vi "onTestDiscovery.vi"(8 "error in (no error)":errorcluster, 11 "Test Runner.Folder in":refnum<class "Test Runner.Folder.lvclass">) -> (0 "error out":errorcluster, 2 "Tests VIs":path[](array[path]), 3 "Test Runner.Folder out":refnum<class "Test Runner.Folder.lvclass">)   [LabVIEW 2020, in "Caraya.lvlib" / "Test Runner.Folder.lvclass"]
uses:
  Test Runner.Folder.lvclass
  Test Runner.Folder.lvclass/Test Runner.Folder.ctl
  <userlib>/_OpenG.lib/file/file.llb/openg_file.lvlib
  <userlib>/_OpenG.lib/file/file.llb/File Exists - Scalar__ogtk.vi
  Test Runner/Test Runner.lvclass
  <userlib>/_OpenG.lib/file/file.llb/Build Path - File Names Array__ogtk.vi
  <userlib>/_OpenG.lib/file/file.llb/File Exists - Array__ogtk.vi
  <userlib>/_OpenG.lib/file/file.llb/Valid Path - Traditional__ogtk.vi
  C:/projects/caraya/src/classes/Test Runner/Test Runner.lvclass
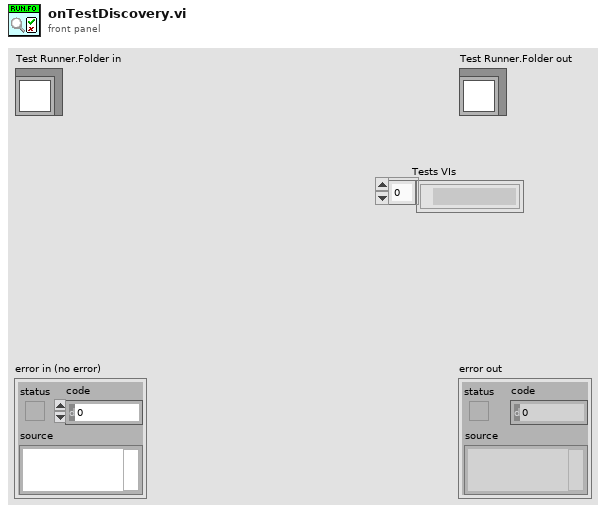
[diagram p1: front panel]
types:
  T1 = typedef "NI_FileType.lvlib/LVFileType.ctl" = enum32{"Invalid file", "Unknown type", "Instrument", "Control", "Polymorphic VI", "Project", "Library", "LVClass", "XControl", "XNode", "Shared library", ".NET assembly", "ActiveX interface", "CIN", "Run-time menu", "Palette menu", "Help file", "LLB", "XNode Edit Dependency", "Class Private Data Control", "Statechart", "MathScript .m file", "Ladder Diagram", "LVLibp", "XNode Build Dependency"}
  T2 = cluster{"path":path, "delimited name":string, "type":T1, "iState":u32, "iStyle":u16, "wStyle":u16, "buttons":u16, "viflags":u32, "viflags2":u32, "links":u32[]}[]
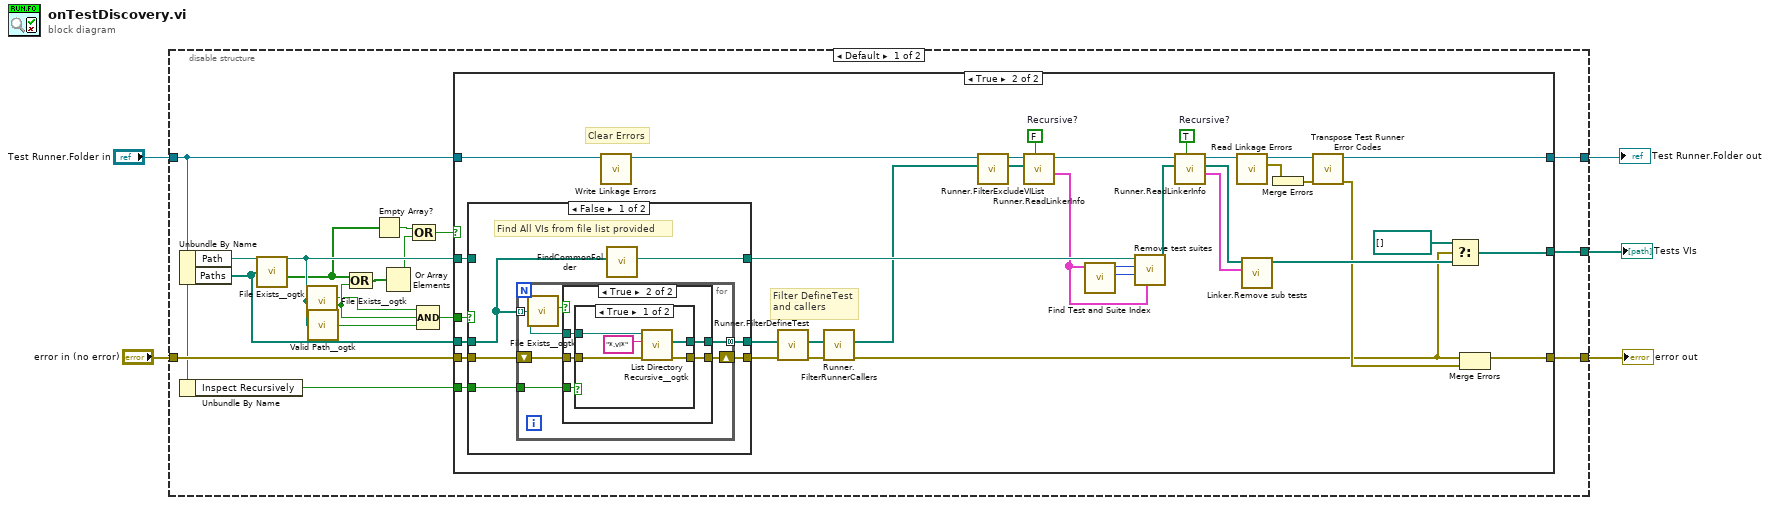
[diagram p0: block diagram]
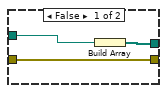
[diagram p3: hidden frame]
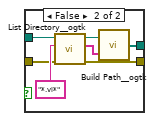
[diagram p4: hidden frame]
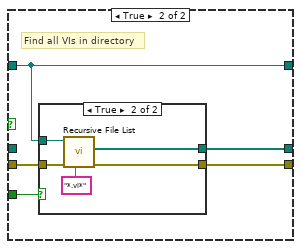
[diagram p5: hidden frame]
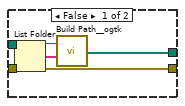
[diagram p6: hidden frame]
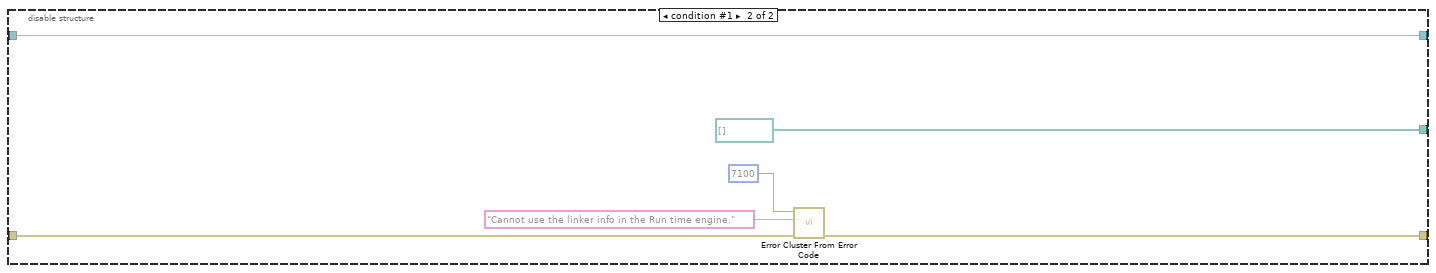
[diagram p7: hidden frame]
diagram:
  n1 = disable-structure shown="Default" {
    disable-tunnel: [w20 w108] -> w2
    disable-tunnel: "Test Runner.Folder in" -> [w16 w107]
    disable-tunnel: [w19 w107] -> w4
    disable-tunnel: [w18 path[] [] ("Test VIs")] -> w3
    disable-tunnel: "error in (no error)" -> [w17 w105]
    frame condition #0 (active) {
      n2 = Unbundle By Name(w16) -> ("Path"=w21:path, "Paths"=w11:path[])
      n3 = Unbundle By Name(w16) -> ("Inspect Recursively"=w15:bool)
      n4 = call-poly <userlib>:"File Exists__ogtk.vi"("file paths"=w11) -> ("exists"=w8:bool[])  [unwired: 6 in, 1 out]
      n5 = call-poly <userlib>:"File Exists__ogtk.vi"("file path"=w21) -> ("is directory"=w13:bool, "exists"=w14:bool)  [unwired: 6 in]
      n6 = call-poly <userlib>:"Valid Path__ogtk.vi"("path"=w21) -> ("valid"=w22:bool)
      n7 = Compound Arithmetic op=OR(w8, w14) -> (w10:bool[])
      n8 = Empty Array?(array=w8) -> (empty?=w9:bool)
      n9 = Or Array Elements(Boolean array=w10) -> (logical OR=w7:bool)
      n10 = Compound Arithmetic op=OR(w9, w7) -> (w6:bool)
      n11 = Compound Arithmetic op=AND(w13, w14, w22) -> (w12:bool)
      n12 = case shown="True" w6 {
        tunnel: w15 -> [_ w57]
        tunnel: [w23 w35] -> w20
        tunnel: [_ w56] -> w18
        tunnel: w21 -> [_ w55]
        tunnel: w16 -> [w24 w44]
        tunnel: [w24 w31] -> w19
        tunnel: w17 -> [w23 w54]
        tunnel: w12 -> [_ w49]
        tunnel: w11 -> [_ w47]
        frame False {
        }
        frame True {
          w41 = TRUE  # Recursive?
          w43 = FALSE  # Recursive?
          # "Filter DefineTest\nand callers"
          # "Clear Errors"
          n13 = case shown="False" w49 {
            tunnel: w57 -> [w58 w94]
            tunnel: w55 -> [_ w90]
            tunnel: w54 -> [w61 w93]
            tunnel: [w60 w92] -> w29
            tunnel: [w59 w91] -> w45
            tunnel: [w63 w90] -> w48
            tunnel: w47 -> [w62 _]
            frame False {
              # "Find All VIs from file list provided"
              n14 = for {
                tunnel: w62 -> [w68] mode=indexing
                shift-right: [w65] -> w60
                shift-left: w61 -> [w66]
                tunnel: [w67] -> w59 mode=concatenating
                tunnel: w58 -> [w64]
                n15 = call-poly <userlib>:"File Exists__ogtk.vi"("file path"=w68) -> ("is directory"=w69:bool)  [unwired: 6 in, 1 out]
                n16 = case shown="True" w69 {
                  tunnel: w68 -> [w72 w76]
                  tunnel: [w71 w75] -> w67
                  tunnel: w66 -> [w70 w73]
                  tunnel: [w70 w74] -> w65
                  tunnel: w64 -> [_ w77]
                  frame False {
                    n17 = Build Array(w72) -> (w71:path[])
                  }
                  frame True {
                    n18 = case shown="True" w77 {
                      tunnel: w76 -> [w82 w89]
                      tunnel: [w81 w83] -> w75
                      tunnel: [w80 w86] -> w74
                      tunnel: w73 -> [w79 w87]
                      frame True {
                        n19 = call <userlib>:"List Directory Recursive__ogtk.vi"("error in (no error)"=w79, "pattern"="*.vi*", "Path"=w82) -> ("error out"=w80:errorcluster, "file paths"=w81:path[])  [unwired: 5 in, 2 out]
                      }
                      frame False {
                        n20 = call <userlib>:"List Directory__ogtk.vi"("error in (no error)"=w87, "pattern"="*.vi*", "directory path"=w89) -> ("error out"=w86:errorcluster, "file names"=w84:string[], "dup directory path"=w85:path)  [unwired: 1 in, 1 out]
                        n21 = call-poly <userlib>:"Build Path__ogtk.vi"("name or relative path"=w84, "base path"=w85) -> ("appended path"=w83:path[])
                      }
                    }
                  }
                }
              }
              n22 = call "FindCommonFolder.vi"("Paths"=w62) -> ("common folder"=w63:path)  [unwired: 10 in]
            }
            frame True {
              # "Find all VIs in directory"
              n23 = case shown="True" w94 {
                tunnel: [w95 w104] -> w91
                tunnel: [w98 w103] -> w92
                tunnel: w90 -> [w99 w102]
                tunnel: w93 -> [_ w100]
                frame False {
                  n24 = List Folder(path=w99) -> (path out=w97:path, filenames=w96:string[], error out=w98:errorcluster)  [unwired: 3 in, 1 out]
                  n25 = call-poly <userlib>:"Build Path__ogtk.vi"("name or relative path"=w96, "base path"=w97) -> ("appended path"=w95:path[])
                }
                frame True {
                  n26 = call <vilib>:"Recursive File List.vi"("pattern"="*.vi*", "error in (no error)"=w100, "Folder Path"=w102) -> ("error out"=w103:errorcluster, "All Files in Dir"=w104:path[])  [unwired: 4 in, 3 out]
                }
              }
            }
          }
          n27 = call "Write Linkage Errors.vi"("Test Runner in"=w44) -> ("Test Runner out"=w28:refnum<class "Test Runner.Folder.lvclass">)  [unwired: 9 in, 1 out]
          n28 = call "Runner.FilterDefineTest.vi"("Paths"=w45) -> ("Filtered Paths"=w46:path[])  [unwired: 10 in]
          n29 = call "Runner.FilterRunnerCallers.vi"("Paths"=w46) -> ("Filtered Paths"=w27:path[])  [unwired: 10 in]
          n30 = call "Runner.FilterExcludeVIList.vi"("Paths"=w27, "Test Runner"=w28) -> ("Filtered Paths"=w26:path[], "Test Runner"=w25:refnum<class "Test Runner.Folder.lvclass">)  [unwired: 8 in]
          n31 = call "Runner.ReadLinkerInfo.vi"("Recursive?"=w43, "VI Paths"=w26, "Test Runner in"=w25) -> ("Linker:Read Info From File"=w42:T2, "Test Runner out"=w37:refnum<class "Test Runner.Folder.lvclass">)  [unwired: 5 in, 2 out]
          n32 = call "Find Test and Suite Index.vi"("Linker.Read Info From File"=w42) -> ("Define Test index"=w52:i32, "Define Test Suite index"=w53:i32)  [unwired: 8 in, 1 out]
          n33 = call "Remove test suites.vi"("Linker.Read Info From File"=w42, "Define Test index"=w52, "Define Test Suite index"=w53, "Directory to search"=w48) -> ("Tests"=w40:path[])  [unwired: 7 in]
          n34 = call "Runner.ReadLinkerInfo.vi"("Recursive?"=w41, "VI Paths"=w40, "Test Runner in"=w37) -> ("Linker:Read Info From File"=w38:T2, "VI Paths (dup)"=w39:path[], "Test Runner out"=w36:refnum<class "Test Runner.Folder.lvclass">)  [unwired: 5 in, 1 out]
          n35 = call "Read Linkage Errors.vi"("Test Runner in"=w36) -> ("Linkage Errors"=w34:errorcluster[], "Test Runner out"=w32:refnum<class "Test Runner.Folder.lvclass">)  [unwired: 8 in, 1 out]
          n36 = call "Linker.Remove sub tests.vi"("Linker.Read Info From File"=w38, "Tests"=w39) -> ("Array"=w51:path[])  [unwired: 9 in]
          n37 = Merge Errors(w34) -> (w33:errorcluster)
          n38 = call-dynamic "Transpose Test Runner Error Codes.vi"("error in (no error)"=w33, "Test Runner in"=w32) -> ("error out"=w30:errorcluster, "Test Runner out"=w31:refnum<class "Test Runner.Folder.lvclass">)  [unwired: 8 in]
          n39 = Select(t=path[] [], s=w29, f=w51) -> (s? t:f=w56:path[])
          n40 = Merge Errors(w29, w30) -> (w35:errorcluster)
        }
      }
    }
    frame condition #1 {
      n41 = call <vilib>:"Error Cluster From Error Code.vi"("error in (no error)"=w105, "error message (\"\")"="Cannot use the linker info in the Run time engine." ("error message (\"\")"), "error code (0)"=7100) -> ("error out"=w108:errorcluster)  [unwired: 6 in]
    }
  }
  "error out" <- w2
  "Test Runner.Folder out" <- w4
  "Tests VIs" <- w3
